vi "query Status Register.vi"(8 "error in (no error)":errorcluster, 11 "FSV-40N in":refnum<class "FSV-40N.lvclass">) -> (0 "error out":errorcluster, 2 "Value (I32)":i32, 3 "FSV-40N out":refnum<class "FSV-40N.lvclass">)   [LabVIEW 2023, in "Spectrum Analyzer.lvlib" / "FSV-40N.lvclass"]
uses:
  FSV-40N.lvclass
  FSV-40N.lvclass/FSV-40N.ctl
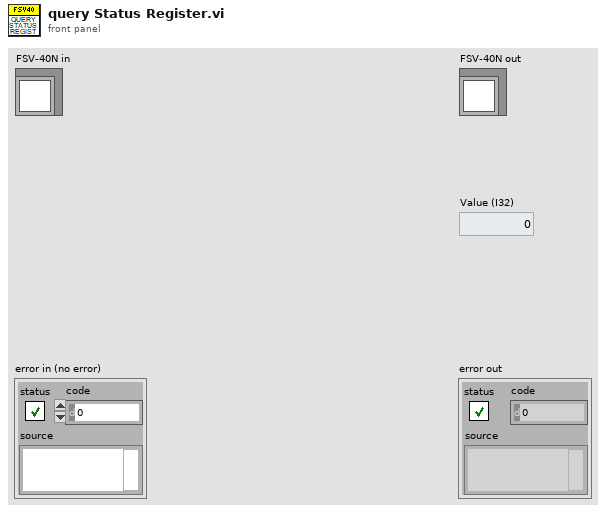
[diagram p1: front panel]
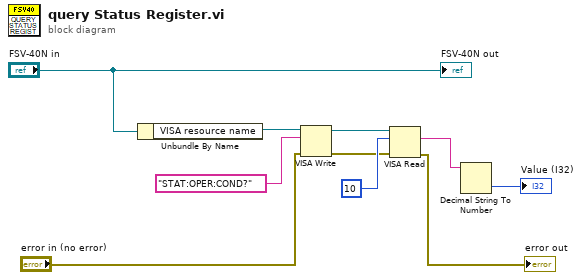
[diagram p0: block diagram]
diagram:
  n1 = Unbundle By Name("FSV-40N in") -> ("VISA resource name"=w9:refnum<visa-resource-name>)
  n2 = VISA Write(VISA resource name=w9, write buffer="STAT:OPER:COND?", error in (no error)="error in (no error)") -> (VISA resource name out=w7:refnum<visa-resource-name>, error out=w5:errorcluster)  [unwired: 1 out]
  n3 = VISA Read(VISA resource name=w7, byte count=u32 10, error in (no error)=w5) -> (read buffer=w4:string, error out=→"error out":errorcluster)  [unwired: 2 out]
  n4 = Decimal String To Number(string=w4) -> (number=→"Value (I32)":i32)  [unwired: 2 in, 1 out]
  "FSV-40N out" <- "FSV-40N in"
